vi "Parse Load SA Level Setting.vi"(8 "error in (no error)":errorcluster caption="에러 입력(에러 없음)", 10 "JSON string":string, 11 "Instrument Manager 입력":refnum<class "Instrument Manager.lvclass">) -> (0 "error out":errorcluster caption="에러 출력", 1 "SA Level Param":T1, 2 "Load SA Level Settting Param":T2, 3 "Instrument Manager 출력":refnum<class "Instrument Manager.lvclass">)   [LabVIEW 2023, in "Instrument Manager.lvclass"]
uses:
  Instrument Manager.lvclass
  Param Definition/Load SA Level Setting Param.ctl
  Type Definition/SA Level Param.ctl
  Instrument Manager.lvclass/Instrument Manager.ctl
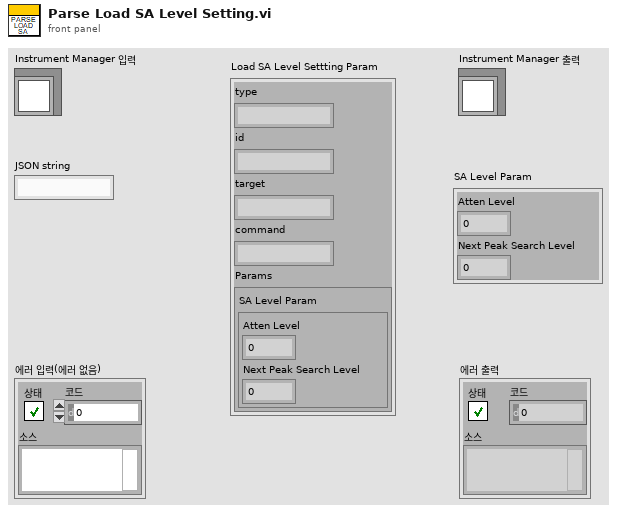
[diagram p1: front panel]
types:
  T1 = typedef "SA Level Param.ctl" = cluster{"Atten Level":dbl, "Next Peak Search Level":dbl}
  T2 = typedef "Instrument Manager.lvclass/Load SA Level Setting Param.ctl" = cluster{"type":string, "id":string, "target":string, "command":string, "Params":cluster{"SA Level Param":T1}}
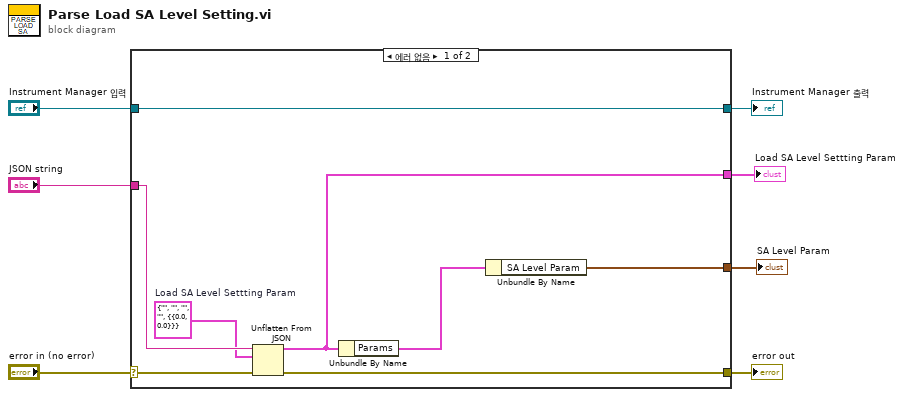
[diagram p0: block diagram]
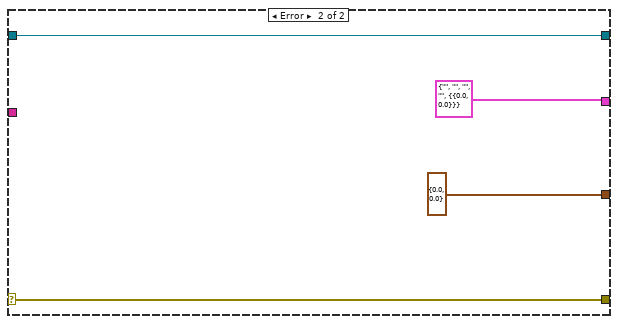
[diagram p2: hidden frame]
diagram:
  n1 = case shown="에러 없음" "error in (no error)" {
    selector: "error in (no error)" -> [w14 w19]
    tunnel: [w9 w19] -> w6
    tunnel: [w8 w18] -> w4
    tunnel: "Instrument Manager 입력" -> [w8 w18]
    tunnel: "JSON string" -> [w15 _]
    tunnel: [w12 T2 {"type"="", "id"="", "target"="", "command"="", "Params"={"SA Level Param"={"Atten Level"=0.0, "Next Peak Search Level"=0.0}}} ("Load SA Level Settting Param")] -> w2
    tunnel: [w10 T1 {"Atten Level"=0.0, "Next Peak Search Level"=0.0} ("SA Level Param")] -> w1
    frame No Error {
      w13 = T2 {"type"="", "id"="", "target"="", "command"="", "Params"={"SA Level Param"={"Atten Level"=0.0, "Next Peak Search Level"=0.0}}}  # Load SA Level Settting Param
      n2 = Unflatten From JSON(JSON string=w15, type and defaults=w13, error in (no error)=w14) -> (value=w12:T2, error out=w9:errorcluster)  [unwired: 4 in]
      n3 = Unbundle By Name(w12) -> ("Params"=w11:cluster{"SA Level Param":T1})
      n4 = Unbundle By Name(w11) -> ("SA Level Param"=w10:T1)
    }
    frame Error {
    }
  }
  "error out" <- w6
  "Instrument Manager 출력" <- w4
  "SA Level Param" <- w1
  "Load SA Level Settting Param" <- w2
